vi "Acquire Data.vi"(7 "user event":T2, 8 "error in (no error)":errorcluster, 9 "UI Refs":T1, 10 "Waveforms":waveform(dbl)[](array[waveform]), 11 "F18 Blowdown":refnum<class "F18 Blowdown.lvclass">) -> (0 "error out":errorcluster, 3 "F18 Blowdown out":refnum<class "F18 Blowdown.lvclass">)   [LabVIEW 2025, in "F18 Blowdown.lvlib" / "F18 Blowdown.lvclass"]
uses:
  F18 Blowdown.lvclass
  Users/Public/Documents/Sandia National Labs/TSS Plugin/CEF.lvlibp/Node/UserEventRef.ctl
  F18 Blowdown.lvclass/F18 Blowdown.ctl
  Users/Public/Documents/Sandia National Labs/TSS Plugin/Tests/XY Plotter.lvlibp/XY  Plotter/XY Plotter.lvclass
  Users/Public/Documents/Sandia National Labs/TSS Plugin/CEF.lvlibp/Node/CEF_Node.lvclass
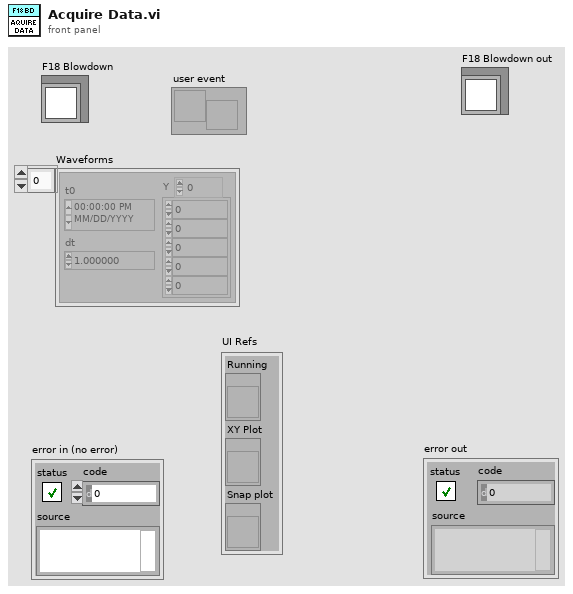
[diagram p1: front panel]
types:
  T1 = cluster{"Running":refnum<vi>, "XY Plot":refnum<vi>, "Snap plot":refnum<vi>}
  T2 = typedef "CEF.lvlibp/CEF_Node.lvclass/UserEventRef.ctl" = refnum<user-event>
  T3 = enum16{"Start Timer", "Read Time", "Pause", "Resume"}
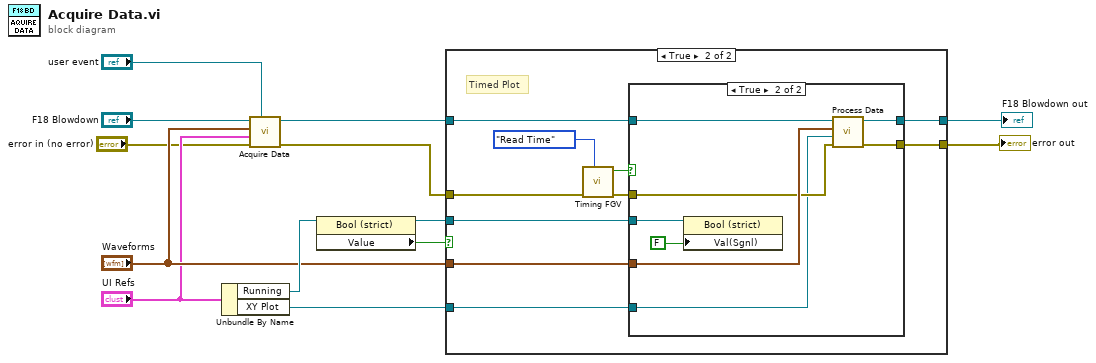
[diagram p0: block diagram]
diagram:
  n1 = Unbundle By Name("UI Refs") -> ("Running"=w8:refnum<vi>, "XY Plot"=w7:refnum<vi>)
  n2 = call-parent "Acquire Data.vi"("user event"="user event", "error in (no error)"="error in (no error)", "UI Refs"="UI Refs", "Waveforms"="Waveforms", "XY Plotter"="F18 Blowdown") -> ("error out"=w1:errorcluster, "XY Plotter out"=w6:refnum<class "F18 Blowdown.lvclass">)  [unwired: 5 in]
  n3 = property class="Bool (strict)"(reference=w8) -> (reference out=w12:refnum<vi>, "Value"=w13:bool)  [unwired: 1 in, 1 out]
  n4 = case shown="True" w13 {
    tunnel: [w15 w25] -> w10
    tunnel: w12 -> [_ w24]
    tunnel: w6 -> [w15 w21]
    tunnel: [w14 w17] -> w9
    tunnel: "Waveforms" -> [_ w20]
    tunnel: w7 -> [_ w18]
    tunnel: w1 -> [w14 w16]
    frame False {
    }
    frame True {
      # "Timed Plot"
      n5 = call "Timing FGV.vi"("Timer Mode"=T3."Read Time", "Error In"=w16) -> ("Error Out"=w19:errorcluster, "Has Time Elapsed"=w23:bool)  [unwired: 7 in, 1 out]
      n6 = case shown="True" w23 {
        tunnel: [w27 w32] -> w25
        tunnel: w24 -> [_ w34]
        tunnel: w21 -> [w27 w33]
        tunnel: [w26 w29] -> w17
        tunnel: w19 -> [w26 w30]
        tunnel: w20 -> [_ w31]
        tunnel: w18 -> [_ w28]
        frame False {
        }
        frame True {
          n7 = property class="Bool (strict)"(reference=w34, "Val(Sgnl)"=FALSE ("Value")) -> ()  [unwired: 1 in, 2 out]
          n8 = call "Process Data.vi"("error in (no error)"=w30, "XY Plot"=w28, "Waveforms"=w31, "F18 Blowdown"=w33) -> ("error out"=w29:errorcluster, "F18 Blowdown out"=w32:refnum<class "F18 Blowdown.lvclass">)  [unwired: 6 in]
        }
      }
    }
  }
  "error out" <- w9
  "F18 Blowdown out" <- w10
